vi "ReCalc_V2.00.vi"(3 "Berechnen":bool, 4 "Datenspeicher":T3={"Fahrzeugdaten"="mit filter hd 85§$", "Auto-Pfad"="26.04.2024 14:10|C:\\Users\\User\\Dropbox\\Prüfstand\\Kurven\\lui\\105\\beduesung", "Rolle [Inkr/U]"=200, "Rollenumfang [m]"=1.255, "Rollenträgheit [kgm²]"=9.1, "Zündung [Imp/U]"=2.0, "Getriebe [1:]"=7.93, "Reifenumfang [m] "=1.293, "Grossanzeige"=7.725, "Gl. Mittelwert"=25, "Differenzenquotient"=8, 1, "dT [s]"=0.0204081632653061, "Strecke [m]"=365.955776857143, "Lufttemperatur [°C]"=13.1, "Mv: n1 [1/min]"=1.0, "Luftdruck [mbar]"=899.6, "nRolle"=array[1261 elements], "nWelle"=array[1261 elements], "AFR"=array[1261 elements], "EGT"=array[1261 elements], "Übersetzung ermitteln aus"=2, "[s]"=3.0, "Mv: M0 [Nm]"=0.0, "Mv: M1 [Nm]"=0.0, "n vom Gas [1/min]"=8000.0, "dT ungefiltert [s]"=array[1261 elements], [], "Boolesch"=FALSE, "Serielle Schnittstelle"="COM13", "nKuWe/nRolle"=7.725, "v vom Gas [km/h]"=0.0}) -> ()   [LabVIEW 2014]
uses:
  <vilib>/Utility/miscctls.llb/LVPointTypeDef.ctl
  <vilib>/Analysis/3filter.llb/IIR Filter (DBL).vi
  <vilib>/Analysis/NI_AALBase.lvlib
panel:
  out "Fahrzeugdaten":string
  out "Ergebnis":string
  out "EGT [°C]":dbl format="%#.1f"
  out "AFR / l":dbl format="%#.1f"
  out "PM-Graph":cluster{dbl[], dbl[]}[](graph)
  in  "AFR, EGT":bool caption="Messung Klimadaten"
  in  "Lambda":bool caption="Messung Klimadaten"
  in  "Überschrift Leistungsdiagramm":string
  out "AFR,EGT-Graph":cluster{dbl[], "AFR":dbl[]}[](graph)
  out "Strecken":T1 {"Strecke7" scale=0.0..500.0; "Strecke6" scale=0.0..500.0; "Strecke5" scale=0.0..500.0; "Strecke4" scale=0.0..500.0; "Strecke3" scale=0.0..500.0; "Strecke2" scale=0.0..500.0; "Strecke1" max=600.0 scale=0.0..500.0}
  out "Dateiname":string
  out "Datum+Zeit":string="26.04.2024 14:10"
  out "Ereigniswert Überlagern":dbl=24.0
  in  "Mv: M1 [Nm]":dbl min=0.0
  in  "Mv: M0 [Nm]":dbl min=0.0
  in  "Mv: n1 [1/min]":u16=1 min=1
  out "Überlagerung":bool
  out "CursorY2 - Beschriftung":string="M [Nm]"
  out "CursorX - Beschriftung":string="n [1/min]"
  out "M [Nm]":dbl=4550.322600913994 format="%#.1f"
  out "P [PS]":dbl=3885.8131998402705 format="%#.1f"
  out "n [1/min]":dbl=5997.814814814815 caption="n {1/min]" format="%#.0f"
  in  "v vom Gas [km/h]":dbl
  in  "Legende":bool=TRUE
  in  "Überlagern":bool
  out "Übersetzung aus:":T2(ring)=enum."nKuWe / nRolle"
  in  "Speichern":bool
  out "Reifenumfang [m]":dbl=1.293
  out "Getriebe [1:]":dbl=7.93
  out "Zündung [Imp/U]":dbl=2.0
  out "Rollengeber [Inkr/U]":u16=200
  out "Luftdruck [mbar]":dbl=899.6
  out "Lufttemperatur [°C]":dbl=13.1
  in  "Stopp":bool
  in  "Rollenträgheit [kgm²]":dbl=9.1
  in  "Gl. Mittelwert":u8=25
  in  "Differenzenquotient":u8=8
  in  "n vom Gas [1/min]":dbl=8000.0
  out "Rollenumfang [m]":dbl=1.255 format="%.3f"
  out "nKuWe / nRolle":dbl=7.725 format="%.2f"
  in  "Drucken":bool
  out "Pmax":string
  in  "Öffnen":bool
  out "[s]":dbl=3.0
  # "AFR / l &  EGT"
  # "AFR <> l"
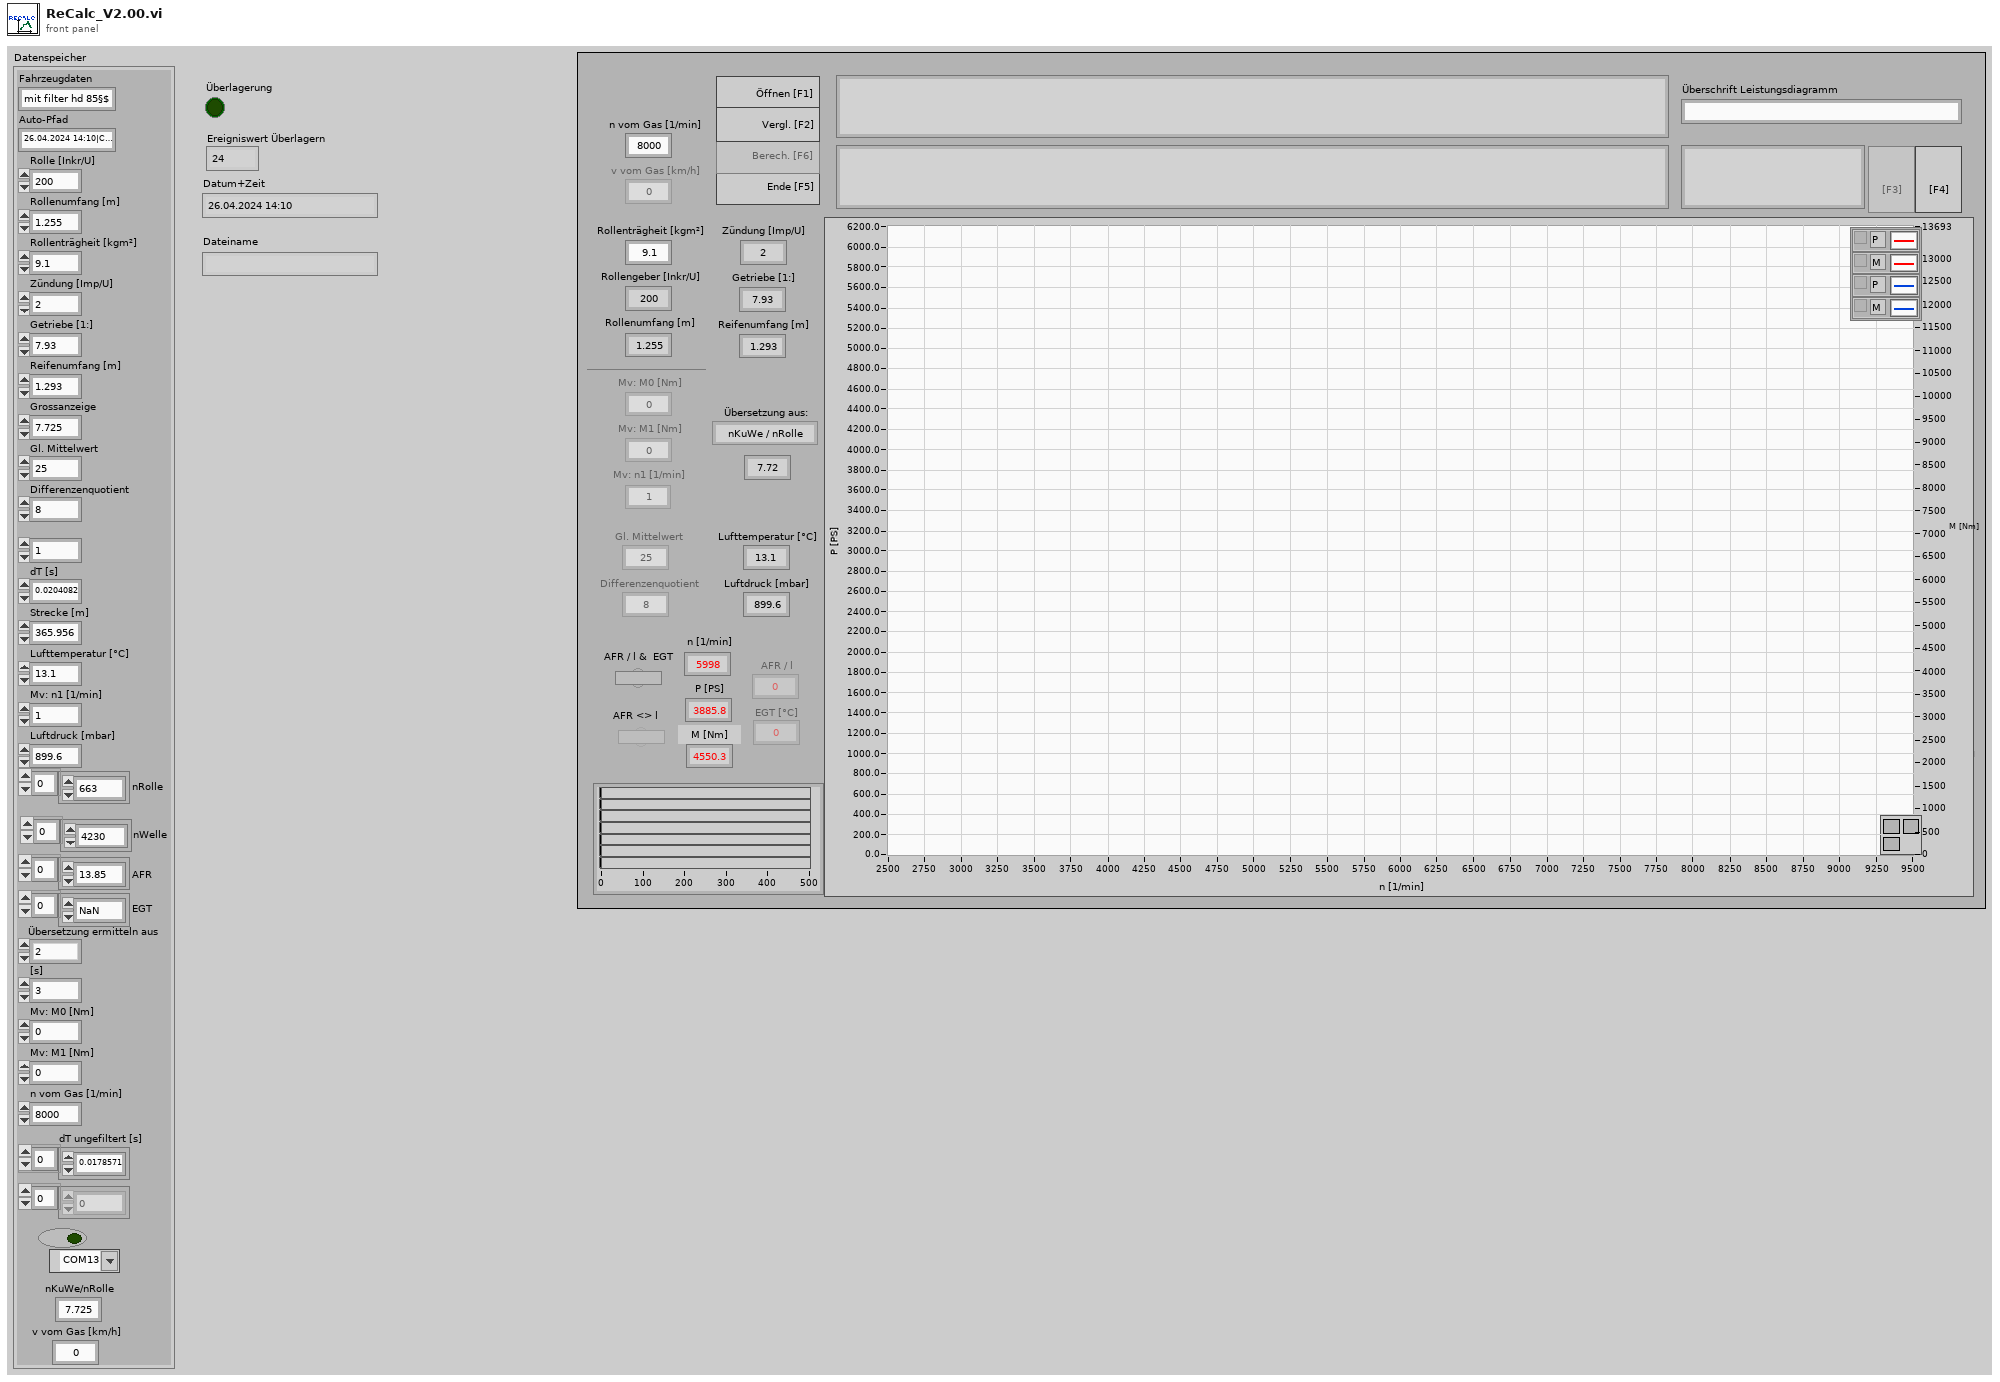
[diagram p1: front panel]
types:
  T1 = cluster{"Strecke1":dbl, "Strecke2":dbl, "Strecke3":dbl, "Strecke4":dbl, "Strecke5":dbl, "Strecke6":dbl, "Strecke7":dbl}
  T2 = enum8{"Zündsignal", "Getriebe & Reifen", "nKuWe / nRolle", "Vario [km/h]"}
  T3 = cluster{"Fahrzeugdaten":string, "Auto-Pfad":string, "Rolle [Inkr/U]":u16, "Rollenumfang [m]":dbl, "Rollenträgheit [kgm²]":dbl, "Zündung [Imp/U]":dbl, "Getriebe [1:]":dbl, "Reifenumfang [m] ":dbl, "Grossanzeige":dbl, "Gl. Mittelwert":u8, "Differenzenquotient":u8, u8, "dT [s]":dbl, "Strecke [m]":dbl, "Lufttemperatur [°C]":dbl, "Mv: n1 [1/min]":dbl, "Luftdruck [mbar]":dbl, "nRolle":dbl[], "nWelle":dbl[], "AFR":dbl[], "EGT":dbl[], "Übersetzung ermitteln aus":u8, "[s]":dbl, "Mv: M0 [Nm]":dbl, "Mv: M1 [Nm]":dbl, "n vom Gas [1/min]":dbl, "dT ungefiltert [s]":dbl[], i32[], "Boolesch":bool, "Serielle Schnittstelle":refnum<visa-resource-name>, "nKuWe/nRolle":dbl, "v vom Gas [km/h]":dbl}
  T4 = typedef "LVPointTypeDef.ctl" = cluster{"Horizontal":i16, "Vertical":i16}
  T5 = enum8{"Enabled", "Disabled", "Disabled and Grayed Out"}
  T6 = cluster{"Fahrzeugdaten":string, "Auto-Pfad":string, "Rolle [Inkr/U]":u16, "Rollenumfang [m]":dbl, "Rollenträgheit [kgm²]":dbl, "Zündung [Imp/U]":dbl, "Getriebe [1:]":dbl, "Reifenumfang [m] ":dbl, "Grossanzeige":dbl, "Gl. Mittelwert":u8, "Differenzenquotient":u8, "AFR,EGT":u8, "dT [s]":dbl, "Strecke [m]":dbl, "Lufttemperatur [°C]":dbl, "Mv: n1 [1/min]":dbl, "Luftdruck [mbar]":dbl, "nRolle":dbl[], "nWelle":dbl[], "AFR":dbl[], "EGT":dbl[], "Übersetzung ermitteln aus":u8, "[s]":dbl, "Mv: M0 [Nm]":dbl, "Mv: M1 [Nm]":dbl, "n vom Gas [1/min]":dbl, "dT-Array [s]":dbl[], i32[], "Boolesch":bool, "Serielle Schnittstelle":refnum<visa-resource-name>, "nKuWe/nRolle":dbl, "v vom Gas [km/h]":dbl}
  T7 = enum16{"Zündsignal", "Getriebe & Reifen", "nKuWe / nRolle", "Vario (km/h)"}
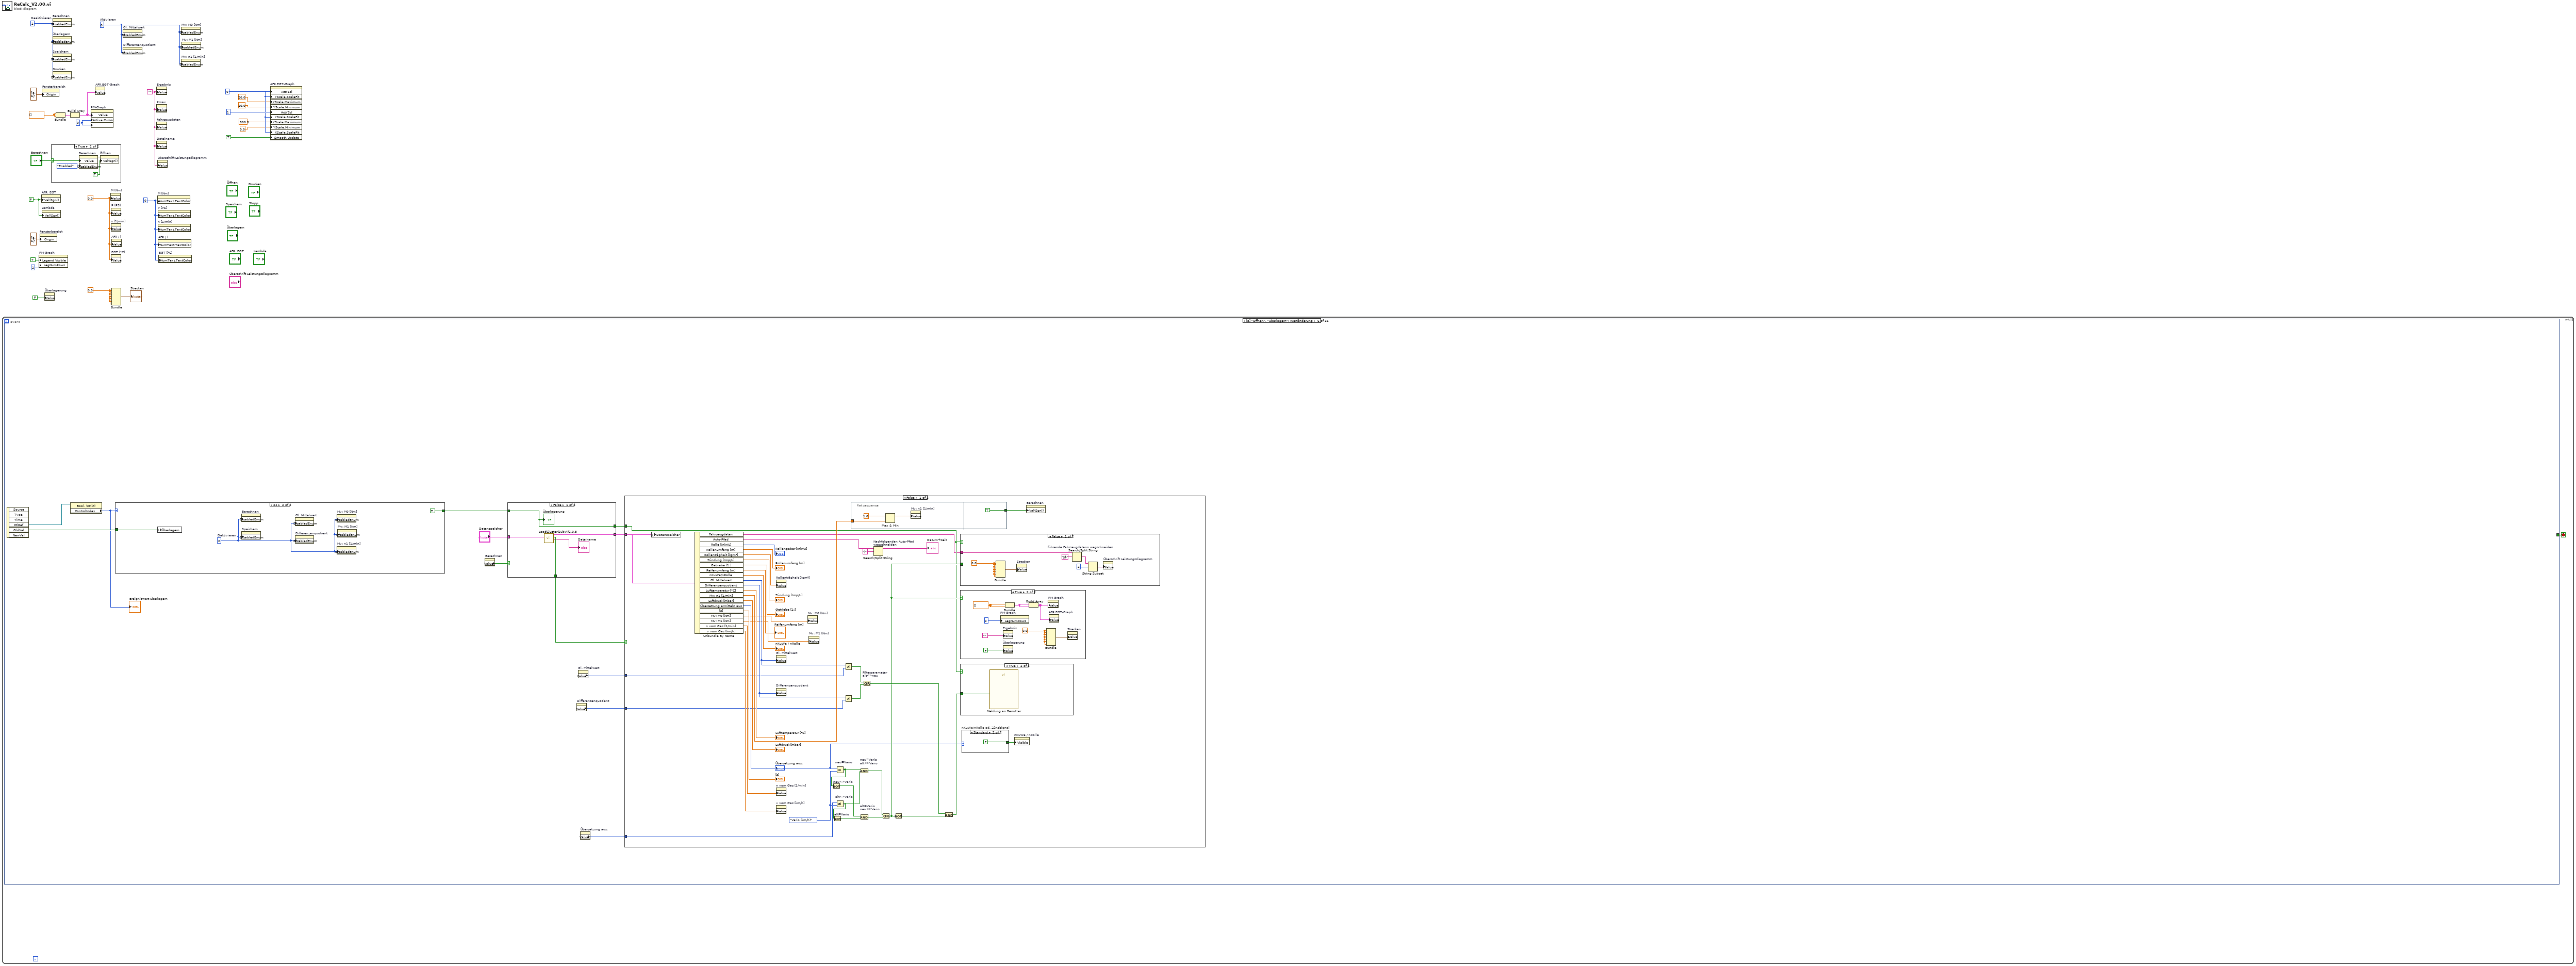
[diagram p0: block diagram]
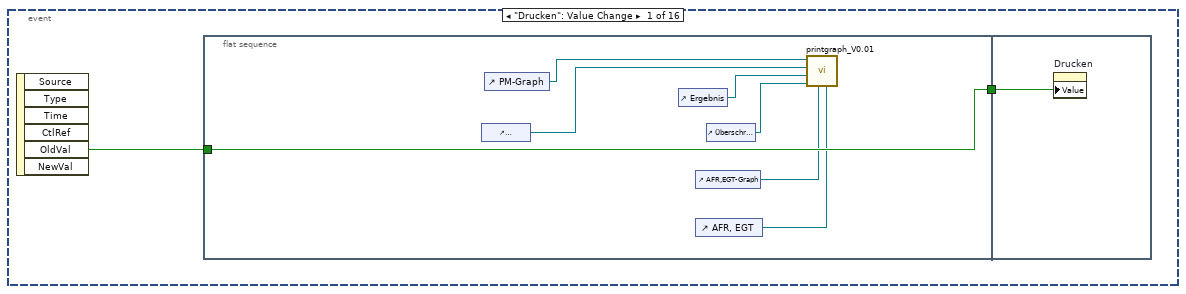
[diagram p3: hidden frame]
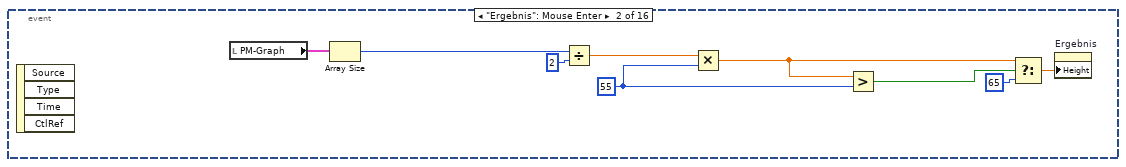
[diagram p4: hidden frame]
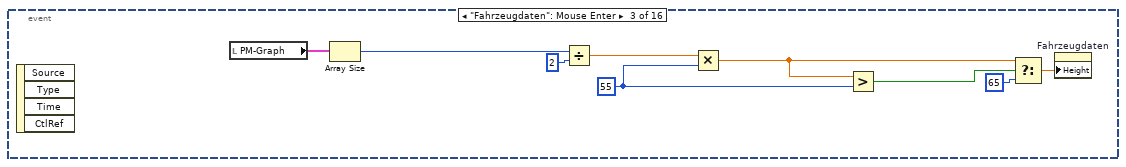
[diagram p5: hidden frame]
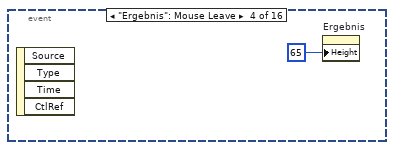
[diagram p6: hidden frame]
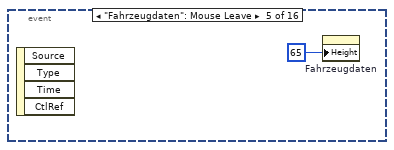
[diagram p7: hidden frame]
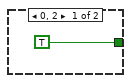
[diagram p8: hidden frame]
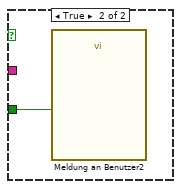
[diagram p10: hidden frame]
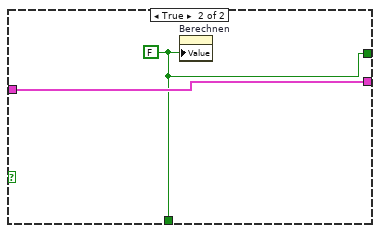
[diagram p13: hidden frame]
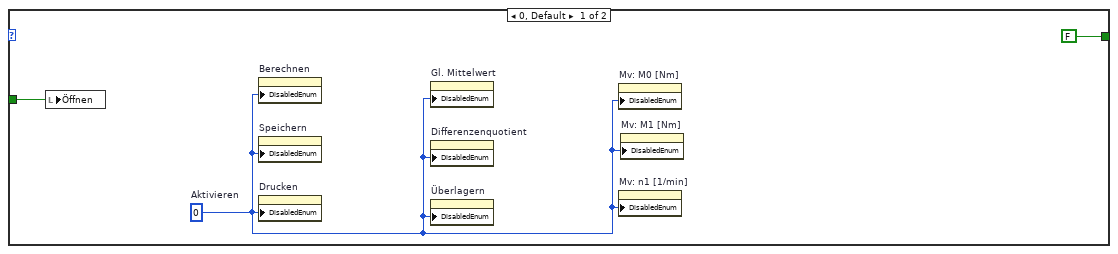
[diagram p14: hidden frame]
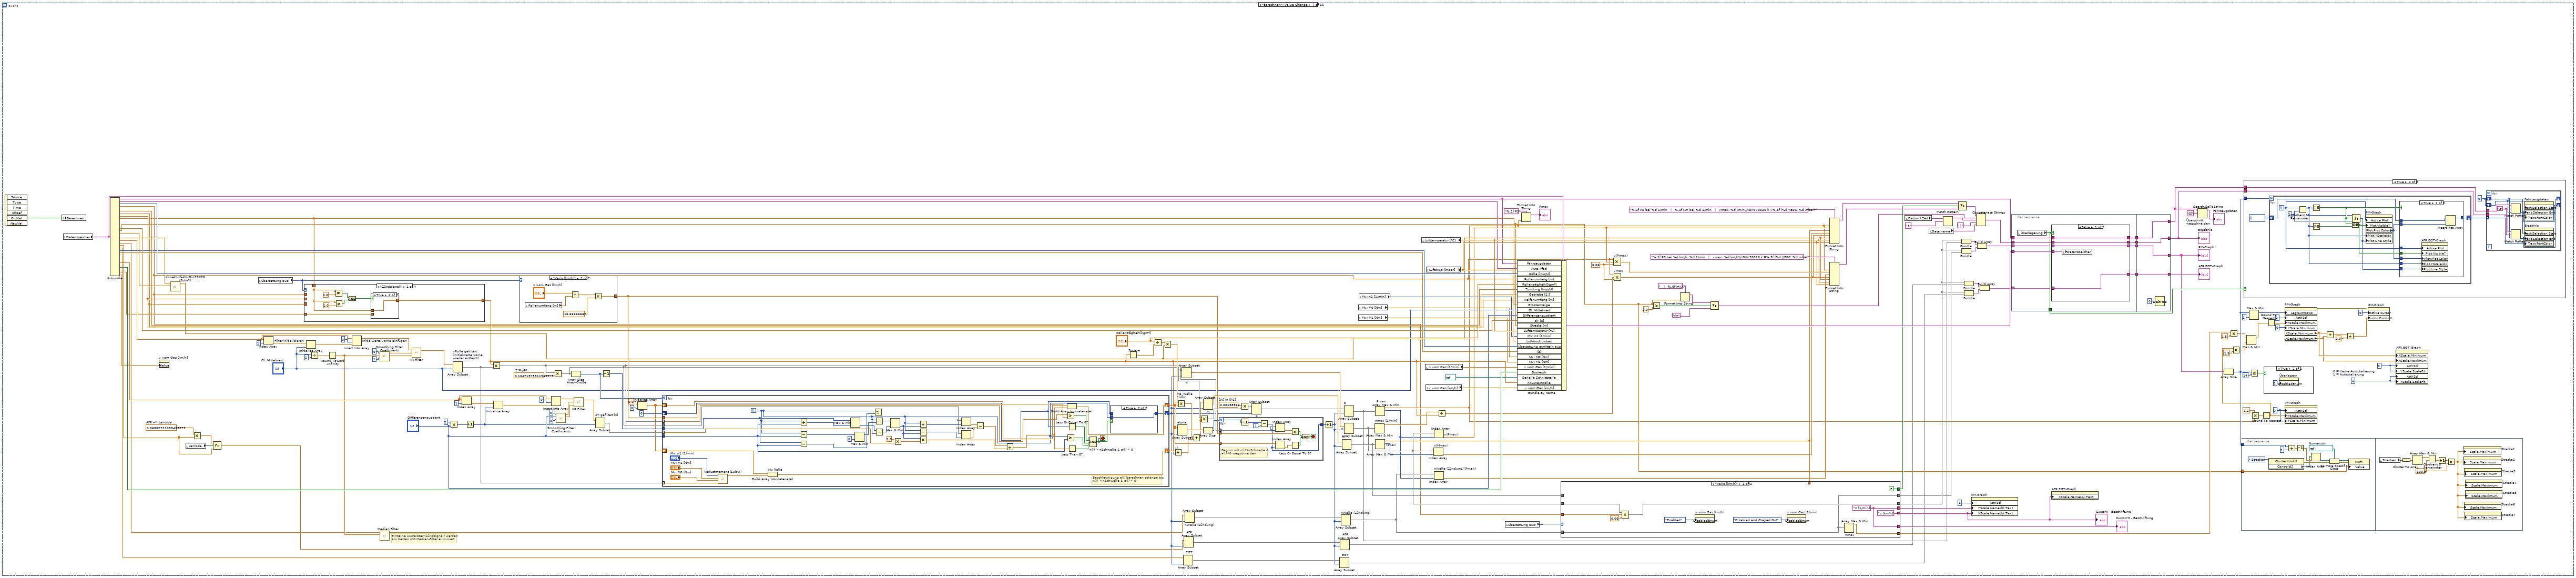
[diagram p15: hidden frame]
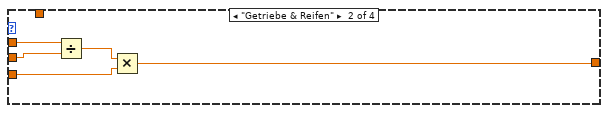
[diagram p17: hidden frame]
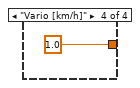
[diagram p19: hidden frame]
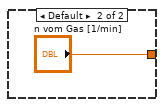
[diagram p20: hidden frame]
diagram:
  w6 = 0
  w10 = FALSE
  w14 = 0.0
  w18 = 0
  w12 = 0
  w11 = 0.0
  w19 = dbl[] []
  w16 = 0  # Aktivieren
  w22 = 2  # Deaktivieren
  w13 = ""
  n1 = while {
    stop <- w26 stop-if-true
    n2 = event shown="[5] \"Öffnen\", \"Überlagern\": Wertänderung" {
      selector: _ -> [_ _ _ _ _ _ _ _ _ _ _ _ _ _ _ _]
      dyn-events: _ -> [_ _ _ _ _ _ _ _ _ _ _ _ _ _ _ _]
      timeout: _ -> [_ _ _ _ _ _ _ _ _ _ _ _ _ _ _ _]
      tunnel: [_ _ _ _ _ _ _ _ w532 _ _ _ _ _ _ _] -> w26
      event "Drucken": Value Change {
        n3 = event-data() -> ("OldVal"=w28:bool)  [unwired: 1 in, 5 out]
        n4 = flat-sequence {
          tunnel: [w35] -> w27
          tunnel: w28 -> [w35]
          tunnel: w27 -> [w36]
          frame #0 {
            n5 = control-ref of="Fahrzeugdaten"() -> (w33:refnum<vi>)
            n6 = control-ref of="PM-Graph"() -> (w34:refnum<vi>)
            n7 = control-ref of="Ergebnis"() -> (w32:refnum<vi>)
            n8 = control-ref of="AFR,EGT-Graph"() -> (w30:refnum<vi>)
            n9 = control-ref of="AFR, EGT"() -> (w29:refnum<vi>)
            n10 = control-ref of="Überschrift Leistungsdiagramm"() -> (w31:refnum<vi>)
            n11 = call "printgraph_V0.01.vi"("AFR"=w29, "AFR-Graph (Eingang)"=w30, "Überschrift"=w31, "Ergebnis"=w32, "Fahrzeugdaten"=w33, "PM-Graph (Eingang)"=w34) -> ()  [unwired: 6 in]
          }
          frame #1 {
            n12 = property on="Drucken" class="Bool. (strikt)"("Value"=w36) -> ()  [unwired: 2 in, 2 out]
          }
        }
      }
      event "Ergebnis": Mouse Enter {
        w39 = u32 55 ("Größe:Höhe")
        n13 = event-data() -> ()  [unwired: 1 in, 4 out]
        n14 = local read "PM-Graph"() -> (w45:cluster{dbl[], dbl[]}[])
        n15 = Array Size(array=w45) -> (size(s)=w44:i32)
        n16 = Divide(x=w44, y=2) -> (x/y=w42:dbl)
        n17 = Multiply(x=w42, y=w39) -> (x*y=w40:dbl)
        n18 = Greater?(x=w40, y=w39) -> (0:w41:bool)
        n19 = Select(t=w40, s=w41, f=u32 65 ("Größe:Höhe")) -> (s? t:f=w38:dbl)
        n20 = property on="Ergebnis" class="Str"("Height"=w38) -> ()  [unwired: 2 in, 2 out]
      }
      event "Fahrzeugdaten": Mouse Enter {
        w48 = u32 55 ("Größe:Höhe")
        n21 = event-data() -> ()  [unwired: 1 in, 4 out]
        n22 = local read "PM-Graph"() -> (w54:cluster{dbl[], dbl[]}[])
        n23 = Array Size(array=w54) -> (size(s)=w53:i32)
        n24 = Divide(x=w53, y=2) -> (x/y=w51:dbl)
        n25 = Multiply(x=w51, y=w48) -> (x*y=w49:dbl)
        n26 = Greater?(x=w49, y=w48) -> (0:w50:bool)
        n27 = Select(t=w49, s=w50, f=u32 65 ("Größe:Höhe")) -> (s? t:f=w47:dbl)
        n28 = property on="Fahrzeugdaten" class="Str"("Height"=w47) -> ()  [unwired: 2 in, 2 out]
      }
      event "Ergebnis": Mouse Leave {
        n29 = event-data() -> ()  [unwired: 1 in, 4 out]
        n30 = property on="Ergebnis" class="Str"("Height"=u32 65 ("Größe:Höhe")) -> ()  [unwired: 2 in, 2 out]
      }
      event "Fahrzeugdaten": Mouse Leave {
        n31 = event-data() -> ()  [unwired: 1 in, 4 out]
        n32 = property on="Fahrzeugdaten" class="Str"("Height"=u32 65 ("Größe:Höhe")) -> ()  [unwired: 2 in, 2 out]
      }
      event "Öffnen", "Überlagern": Value Change {
        n33 = event-data() -> ("CtlRef"=w67:refnum<vi>, "OldVal"=w58:bool)  [unwired: 1 in, 4 out]
        n34 = property class="Bool. (strikt)"(reference=w67) -> ("ControlIndex"=w57:i32)  [unwired: 1 in, 2 out]
        "Ereigniswert Überlagern" <- w57
        n35 = case shown="24" w57 {
          tunnel: w58 -> [w143 w146]
          tunnel: [FALSE ("Überlagerung") TRUE ("Überlagerung")] -> w66
          frame 0, Default {
            w141 = 0  # Aktivieren
            n36 = local write "Öffnen"(w143) -> ()
            n37 = property on="Berechnen" class="Bool. (strikt)"("DisabledEnum"=w141) -> ()  [unwired: 2 in, 2 out]
            n38 = property on="Speichern" class="Bool. (strikt)"("DisabledEnum"=w141) -> ()  [unwired: 2 in, 2 out]
            n39 = property on="Drucken" class="Bool. (strikt)"("DisabledEnum"=w141) -> ()  [unwired: 2 in, 2 out]
            n40 = property on="Gl. Mittelwert" class="DigWert (strikt)"("DisabledEnum"=w141) -> ()  [unwired: 2 in, 2 out]
            n41 = property on="Differenzenquotient" class="DigWert (strikt)"("DisabledEnum"=w141) -> ()  [unwired: 2 in, 2 out]
            n42 = property on="Überlagern" class="Bool. (strikt)"("DisabledEnum"=w141) -> ()  [unwired: 2 in, 2 out]
            n43 = property on="Mv: M0 [Nm]" class="DigWert (strikt)"("DisabledEnum"=w141) -> ()  [unwired: 2 in, 2 out]
            n44 = property on="Mv: n1 [1/min]" class="DigWert (strikt)"("DisabledEnum"=w141) -> ()  [unwired: 2 in, 2 out]
            n45 = property on="Mv: M1 [Nm]" class="DigWert (strikt)"("DisabledEnum"=w141) -> ()  [unwired: 2 in, 2 out]
          }
          frame 24 {
            w144 = 2  # Dektivieren
            n46 = local write "Überlagern"(w146) -> ()
            n47 = property on="Berechnen" class="Bool. (strikt)"("DisabledEnum"=w144) -> ()  [unwired: 2 in, 2 out]
            n48 = property on="Speichern" class="Bool. (strikt)"("DisabledEnum"=w144) -> ()  [unwired: 2 in, 2 out]
            n49 = property on="Gl. Mittelwert" class="DigWert (strikt)"("DisabledEnum"=w144) -> ()  [unwired: 2 in, 2 out]
            n50 = property on="Differenzenquotient" class="DigWert (strikt)"("DisabledEnum"=w144) -> ()  [unwired: 2 in, 2 out]
            n51 = property on="Mv: M0 [Nm]" class="DigWert (strikt)"("DisabledEnum"=w144) -> ()  [unwired: 2 in, 2 out]
            n52 = property on="Mv: n1 [1/min]" class="DigWert (strikt)"("DisabledEnum"=w144) -> ()  [unwired: 2 in, 2 out]
            n53 = property on="Mv: M1 [Nm]" class="DigWert (strikt)"("DisabledEnum"=w144) -> ()  [unwired: 2 in, 2 out]
          }
        }
        n54 = property on="Berechnen" class="Bool. (strikt)"() -> ("Value"=w65:bool)  [unwired: 2 in, 2 out]
        n55 = case shown="False" w65 {
          tunnel: "Datenspeicher" -> [w137 w140]
          tunnel: w66 -> [w138 _]
          tunnel: [w136 w140] -> w63
          tunnel: [w138 w139] -> w64
          tunnel: [w135 w139] -> w62
          frame False {
            n56 = call "LoadCluster(SubVI)2.0.5.vi"("Datenspeicher"=w137) -> ("Dateiname"=→"Dateiname":string, "cancelled"=w135:bool, "Value"=w136:T6)  [unwired: 8 in]
            "Überlagerung" <- w138
          }
          frame True {
            w139 = FALSE
            n57 = property on="Berechnen" class="Bool. (strikt)"("Value"=w139) -> ()  [unwired: 2 in, 2 out]
          }
        }
        n58 = property on="Differenzenquotient" class="DigWert (strikt)"() -> ("Value"=w60:u8)  [unwired: 2 in, 2 out]
        n59 = property on="Gl. Mittelwert" class="DigWert (strikt)"() -> ("Value"=w59:u8)  [unwired: 2 in, 2 out]
        n60 = property on="Übersetzung aus:" class="Enum (strikt)"() -> ("Value"=w61:T2)  [unwired: 2 in, 2 out]
        n61 = case shown="False" w62 {
          tunnel: w64 -> [w88 _]
          tunnel: w63 -> [w90 _]
          tunnel: w61 -> [w81 _]
          tunnel: w60 -> [w80 _]
          tunnel: w59 -> [w79 _]
          frame False {
            w82 = T7."Vario (km/h)"
            n62 = local write "Datenspeicher"(w90) -> ()
            n63 = Unbundle By Name(w90) -> ("Fahrzeugdaten"=w71:string, "Auto-Pfad"=w74:string, "Rolle [Inkr/U]"=→"Rollengeber [Inkr/U]":u16, "Rollenumfang [m]"=→"Rollenumfang [m]":dbl, "Rollenträgheit [kgm²]"=w102:dbl, "Zündung [Imp/U]"=→"Zündung [Imp/U]":dbl, "Getriebe [1:]"=→"Getriebe [1:]":dbl, "Reifenumfang [m]"=→"Reifenumfang [m]":dbl, "nKuWe/nRolle"=→"nKuWe / nRolle":dbl, "Gl. Mittelwert"=w99:u8, "Differenzenquotient"=w98:u8, "Lufttemperatur [°C]"=→"Lufttemperatur [°C]":dbl, "Mv: n1 [1/min]"=w108:dbl, "Luftdruck [mbar]"=→"Luftdruck [mbar]":dbl, "Übersetzung ermitteln aus"=w70:u8, "[s]"=→"[s]":dbl, "Mv: M0 [Nm]"=w76:dbl, "Mv: M1 [Nm]"=w75:dbl, "n vom Gas [1/min]"=w110:dbl, "v vom Gas [km/h]"=w94:dbl)
            "Übersetzung aus:" <- w70
            n64 = property on="Rollenträgheit [kgm²]" class="DigWert (strikt)"("Value"=w102) -> ()  [unwired: 2 in, 2 out]
            n65 = property on="Gl. Mittelwert" class="DigWert (strikt)"("Value"=w99) -> ()  [unwired: 2 in, 2 out]
            n66 = property on="Differenzenquotient" class="DigWert (strikt)"("Value"=w98) -> ()  [unwired: 2 in, 2 out]
            n67 = property on="n vom Gas [1/min]" class="DigWert (strikt)"("Value"=w110) -> ()  [unwired: 2 in, 2 out]
            n68 = property on="v vom Gas [km/h]" class="DigWert (strikt)"("Value"=w94) -> ()  [unwired: 2 in, 2 out]
            n69 = property on="Mv: M0 [Nm]" class="DigWert (strikt)"("Value"=w76) -> ()  [unwired: 2 in, 2 out]
            n70 = property on="Mv: M1 [Nm]" class="DigWert (strikt)"("Value"=w75) -> ()  [unwired: 2 in, 2 out]
            n71 = Equal? "neu=Vario"(x=w70, y=w82) -> (x = y?=w83:bool)
            n72 = Not "neu<>Vario"(x=w83) -> (.not. x?=w84:bool)
            n73 = Not Equal? "alt<>Vario"(x=w81, y=w82) -> (x != y?=w77:bool)
            n74 = Not "alt=Vario"(x=w77) -> (.not. x?=w78:bool)
            n75 = Not Equal?(x=w99, y=w79) -> (x != y?=w97:bool)
            n76 = Not Equal?(x=w98, y=w80) -> (x != y?=w96:bool)
            n77 = flat-sequence {
              tunnel: w108 -> [w132]
              tunnel: [TRUE] -> w91
              frame #0 {
                n78 = Max & Min(x=1.0, y=w132) -> (max(x,y)=w130:dbl)  [unwired: 1 out]
                n79 = property on="Mv: n1 [1/min]" class="DigWert (strikt)"("Value"=w130) -> ()  [unwired: 2 in, 2 out]
              }
              frame #1 {
              }
            }
            n80 = And "neu=Vario\nalt<>Vario"(x=w83, y=w77) -> (x .and. y?=w86:bool)
            n81 = And "alt=Vario\nneu<>Vario"(x=w84, y=w78) -> (x .and. y?=w85:bool)
            n82 = Or "Filterparameter\nalt<>neu"(x=w97, y=w96) -> (x .or. y?=w92:bool)
            n83 = Search/Split String "Nachfolgenden Auto-Pfad wegschneiden"(string=w74, search string/char (-)="|") -> (substring before match=→"Datum+Zeit":string)  [unwired: 1 in, 2 out]
            n84 = Or(x=w86, y=w85) -> (x .or. y?=w89:bool)
            n85 = Not(x=w89) -> (.not. x?=w93:bool)
            n86 = And(x=w92, y=w93) -> (x .and. y?=w87:bool)
            n87 = case shown="True" w89 {
              frame False {
              }
              frame True {
                w116 = 0.0
                w117 = dbl[] []
                n88 = property on="PM-Graph" class="XYGraph (strikt)"("LegNumRows"=2) -> ()  [unwired: 2 in, 2 out]
                n89 = property on="Ergebnis" class="Str"("Value"="") -> ()  [unwired: 2 in, 2 out]
                n90 = property on="Überlagerung" class="Bool. (strikt)"("Value"=FALSE) -> ()  [unwired: 2 in, 2 out]
                n91 = Bundle(w117, w117) -> (w114:cluster{dbl[], dbl[]})  [unwired: 1 in]
                n92 = Build Array(w114, w114) -> (w113:cluster{dbl[], dbl[]}[])
                n93 = Bundle(w116, w116, w116, w116, w116, w116, w116) -> (w115:cluster{dbl, dbl, dbl, dbl, dbl, dbl, dbl})  [unwired: 1 in]
                n94 = property on="PM-Graph" class="XYGraph (strikt)"("Value"=w113) -> ()  [unwired: 2 in, 2 out]
                n95 = property on="AFR,EGT-Graph" class="XYGraph (strikt)"("Value"=w113) -> ()  [unwired: 2 in, 2 out]
                n96 = property on="Strecken" class="Cluster (strikt)"("Value"=w115) -> ()  [unwired: 2 in, 2 out]
              }
            }
            n97 = case shown="True" w88 {
              tunnel: w87 -> [_ w129]
              frame False {
              }
              frame True {
                n98 = call "Meldung an Benutzer"("Enable"=w129) -> ()  [unwired: 9 in, 2 out]
              }
            }
            n99 = case shown="False" w88 {
              tunnel: w89 -> [_ w128]
              tunnel: w71 -> [w121 _]
              frame False {
                w126 = 0.0
                n100 = Bundle(w126, w126, w126, w126, w126, w126, w126) -> (w127:cluster{dbl, dbl, dbl, dbl, dbl, dbl, dbl})  [unwired: 1 in]
                n101 = property on="Strecken" class="Cluster (strikt)"("Value"=w127) -> ()  [unwired: 2 in, 2 out]
                n102 = Search/Split String "führende Fahrzeugdatenn wegschneiden"(string=w121, search string/char (-)="§$") -> (match + rest of string=w124:string)  [unwired: 1 in, 2 out]
                n103 = String Subset(string=w124, offset (0)=2) -> (substring=w125:string)  [unwired: 1 in]
                n104 = property on="Überschrift Leistungsdiagramm" class="Str"("Value"=w125) -> ()  [unwired: 2 in, 2 out]
              }
              frame True {
                n105 = call "Meldung an Benutzer2"("Enable"=w128) -> ()  [unwired: 9 in, 2 out]
              }
            }
            n106 = case "nKuWe/nRolle od. Zündsignal" shown="Standard" w70 {
              tunnel: [TRUE FALSE] -> w69
              frame 0, 2 {
              }
              frame Default {
              }
            }
            n107 = property on="nKuWe / nRolle" class="DigWert (strikt)"("Visible"=w69) -> ()  [unwired: 2 in, 2 out]
            n108 = property on="Berechnen" class="Bool. (strikt)"("Val(Sgnl)"=w91) -> ()  [unwired: 2 in, 2 out]
          }
          frame True {
          }
        }
      }
      event "Berechnen": Value Change {
        w156 = 0.06802721088435375  # AFR --> Lambda
        w168 = 1  # 0 = Keine Autoskalierung 1 = Autoskalierung
        w169 = 0
        w226 = 0.06
        w180 = 0
        w329 = 0.00135962  # [W] in [PS]
        w335 = 0.10471975511965978  # 2*Pi/60
        # "Einzelne Ausreisser (Zündsignal) werden\nam besten mit Median-Filter eliminiert"
        n109 = event-data() -> ("OldVal"=w304:bool)  [unwired: 1 in, 5 out]
        n110 = local write "Berechnen"(w304) -> ()
        n111 = local read "Datenspeicher"() -> (w311:T3)
        n112 = Unbundle(w311) -> ("Fahrzeugdaten"=w189:string, "Auto-Pfad"=w217:string, "Rolle [Inkr/U]"=w310:u16, "Rollenumfang [m]"=w150:dbl, "Zündung [Imp/U]"=w307:dbl, "Getriebe [1:]"=w148:dbl, "Reifenumfang [m]"=w149:dbl, "Grossanzeige"=w147:dbl, "dT [s]"=w279:dbl, "Strecke [m]"=w190:dbl, "Lufttemperatur [°C]"=w203:dbl, "Luftdruck [mbar]"=w202:dbl, "nRolle"=w244:dbl[], "nWelle"=w233:dbl[], "AFR"=w154:dbl[], "EGT"=w162:dbl[], "Übersetzung ermitteln aus"=w245:u8, "[s]"=w305:dbl, "dT ungefiltert [s]"=w243:dbl[], "Boolesch"=w308:bool, "nKuWe/nRolle"=w151:dbl, "v vom Gas [km/h]"=w264:dbl)  [unwired: 10 out]
        n113 = property on="v vom Gas [km/h]" class="DigWert (strikt)"("Value"=w264) -> ()  [unwired: 2 in, 2 out]
        n114 = call "KorrekturfaktorDin70020 (SubVI).vi"("Lufttemperatur [°C]"=w203, "Luftdruck [mbar]"=w202) -> ("Korrekturfaktor"=w201:dbl)  [unwired: 9 in]
        n115 = local read "Lambda"() -> (w158:bool)
        n116 = Multiply(x=w156, y=w154) -> (x*y=w155:dbl[])
        n117 = Select(t=w155, s=w158, f=w154) -> (s? t:f=w157:dbl[])
        n118 = local read "Übersetzung aus:"() -> (w153:T2)
        n119 = Index Array "Filter initialisieren"(array=w244, index=1) -> (element=w315:dbl)
        n120 = case shown="\"Zündsignal\"" w153 {
          tunnel: [w340 w350 w355 1.0] -> w152
          tunnel: w151 -> [w341 _ w355 _]
          tunnel: w150 -> [_ w354 _ _]
          tunnel: w149 -> [_ w353 _ _]
          tunnel: w148 -> [_ w351 _ _]
          tunnel: w147 -> [w342 _ _ _]
          frame "Zündsignal" {
            n121 = Not Equal?(x=w342, y=0.0) -> (x != y?=w344:bool)
            n122 = Not Equal?(x=w342, y=1.0) -> (x != y?=w345:bool)
            n123 = And(x=w344, y=w345) -> (x .and. y?=w343:bool)
            n124 = case shown="True" w343 {
              tunnel: w342 -> [_ w349]
              tunnel: w341 -> [w348 _]
              tunnel: [w348 w349] -> w340
              frame False {
              }
              frame True {
              }
            }
          }
          frame "Getriebe & Reifen" {
            n125 = Divide(x=w354, y=w353) -> (x/y=w352:dbl)
            n126 = Multiply(x=w352, y=w351) -> (x*y=w350:dbl)
          }
          frame "nKuWe / nRolle" {
          }
          frame "Vario [km/h]" {
          }
        }
        n127 = Initialize Array(w315, "Gl. Mittelwert") -> (w316:dbl[])
        n128 = Divide(x="Gl. Mittelwert", y=2) -> (x/y=w337:dbl)
        n129 = Round Toward -Infinity(1:w337) -> (0:w235:dbl)
        n130 = Insert Into Array "Initialwerte vorne einfügen"(array=w244, index=0, new element=w316) -> (w242:dbl[])
        n131 = call <vilib>:"Smoothing Filter Coefficients.vi"("shape"=1, "half-width"=w235, "type"=0) -> ("forward coefficients"=w246:dbl[], "reverse coefficients"=w247:dbl[])  [unwired: 6 in, 1 out]
        n132 = call <vilib>:"Median Filter.vi"("left rank"=w235, "X"=w233) -> ("Filtered X"=w232:dbl[])  [unwired: 8 in, 1 out]
        n133 = call-poly <vilib>:"IIR Filter.vi"("Forward Coefficients"=w246, "Reverse Coefficients"=w247, "X"=w242) -> ("Filtered X"=w313:dbl[])  [unwired: 1 in, 1 out]
        n134 = Multiply(x=2, y="Differenzenquotient") -> (x*y=w287:i32)
        n135 = Array Subset "nRolle gefiltert\n(Initialwerte vorne \nwieder entfernt)"(array=w313, index="Gl. Mittelwert") -> (w213:dbl[])  [unwired: 1 in]
        n136 = Index Array(array=w243, index=1 ("Index")) -> (element=w285:dbl)
        n137 = Increment(x=w287) -> (x+1=w280:i32)
        n138 = Multiply(x=w152, y=w213) -> (x*y=w237:dbl[])
        n139 = Initialize Array(w285, w280) -> (w283:dbl[])
        n140 = case shown="\"Vario [km/h]\"" w153 {
          tunnel: [w379 "n vom Gas [1/min]"] -> w263
          frame "Vario [km/h]" {
            n141 = local read "Rollenumfang [m]"() -> (w380:dbl)
            n142 = Divide(x="v vom Gas [km/h]", y=w380) -> (x/y=w378:dbl)
            n143 = Multiply(x=w378, y=16.66666667) -> (x*y=w379:dbl)
          }
          frame Default {
          }
        }
        n144 = Insert Into Array(array=w243, index=0 ("Index"), new element=w283) -> (w282:dbl[])
        n145 = Multiply(x=w237, y=w335) -> (x*y=w275:dbl[])
        n146 = call <vilib>:"Smoothing Filter Coefficients.vi"("shape"=0, "half-width"="Differenzenquotient", "type"=0) -> ("forward coefficients"=w290:dbl[], "reverse coefficients"=w291:dbl[])  [unwired: 6 in, 1 out]
        n147 = Array Size "Array-Größe"(array=w275) -> (size(s)=w333:i32)
        n148 = call-poly <vilib>:"IIR Filter.vi"("Forward Coefficients"=w290, "Reverse Coefficients"=w291, "X"=w282) -> ("Filtered X"=w281:dbl[])  [unwired: 1 in, 1 out]
        n149 = Array Subset "dT gefiltert [s]"(array=w281, index=w280) -> (w241:dbl[])  [unwired: 1 in]
        n150 = Decrement(x=w333) -> (x-1=w334:i32)
        n151 = Initialize Array(0.0 ("y"), 0) -> (w212:dbl[])
        n152 = for {
          N: w333 -> [_]
          tunnel: "Differenzenquotient" -> [w508]
          tunnel: w275 -> [w497]
          tunnel: w334 -> [w507]
          shift-right: [w512] -> w276
          shift-left: w212 -> [w496]
          tunnel: w237 -> [w510] mode=indexing
          tunnel: w263 -> [w494]
          shift-right: [w501] -> w160
          shift-left: 0 -> [w493]
          tunnel: w241 -> [w498] mode=indexing
          tunnel: w213 -> [w492] mode=indexing
          shift-right: [w486] -> w211
          shift-left: w212 -> [w487]
          i -> [w495]
          stop <- w502 stop-if-true
          # "Beschleunigung a(i) berechnen solange bis\nn(i) > nSchwelle & a(i) < 0"
          n153 = call "Verlustmoment (SubVI).vi"("n [1/min"=w492, "Verlustmoment M0 [Nm] bei n = 0"="Mv: M0 [Nm]", "Verlustmoment M1 [Nm] bei n1"="Mv: M1 [Nm]", "Rollendrehzahl n1 [1/min]"="Mv: n1 [1/min]") -> ("Mv"=w488:dbl)  [unwired: 7 in]
          n154 = Build Array (concatenate) "Mv Rolle"(w487, w488) -> (w486:dbl[])
          n155 = Add(x=w495, y=w508) -> (x+y=w520:i32)
          n156 = Subtract(x=w495, y=w508) -> (x-y=w526:i32)
          n157 = Subtract(x=w507, y=w508) -> (x-y=w509:i32)
          n158 = Max & Min(x=w507, y=w520) -> (min(x,y)=w521:i32)  [unwired: 1 out]
          n159 = Max & Min(x=w526, y=0) -> (max(x,y)=w524:i32)  [unwired: 1 out]
          n160 = Less Or Equal?(x=w495, y=w509) -> ()  [unwired: 1 out]
          n161 = Subtract(x=w495, y=w524) -> (x-y=w523:i32)
          n162 = Subtract(x=w521, y=w495) -> (x-y=w522:i32)
          n163 = Max & Min(x=w523, y=w522) -> (min(x,y)=w514:i32)  [unwired: 1 out]
          n164 = Multiply(x=2.0, y=w498) -> (x*y=w499:dbl)
          n165 = Add(x=w495, y=w514) -> (x+y=w519:i32)
          n166 = Subtract(x=w495, y=w514) -> (x-y=w518:i32)
          n167 = Multiply(x=w514, y=w499) -> (x*y=w513:dbl)
          n168 = Index Array(array=w497, index=w519) -> (element=w516:dbl)
          n169 = Index Array(array=w497, index=w518) -> (element=w517:dbl)
          n170 = Subtract(x=w516, y=w517) -> (x-y=w515:dbl)
          n171 = Divide(x=w515, y=w513) -> (x/y=w506:dbl)
          n172 = Greater?(x=w510, y=w494) -> (0:w511:bool)
          n173 = Greater Or Equal?(x=w495, y=w508) -> (x >= y?=w505:bool)
          n174 = Build Array (concatenate)(w496, w506) -> (w512:dbl[])
          n175 = Less Or Equal To 0?(x=w493) -> (x <= 0?=w503:bool)
          n176 = Less Than 0?(x=w506) -> (x < 0?=w504:bool)
          n177 = Compound Arithmetic op=AND "n(i) > nSchwelle & a(i) < 0"(w504, w511, w503, w505) -> (w502:bool)
          n178 = case shown="True" w502 {
            tunnel: w495 -> [_ w528]
            tunnel: [w527 w528] -> w501
            tunnel: w493 -> [w527 _]
            frame False {
            }
            frame True {
            }
          }
        }
        n179 = Square(x=w152) -> (x^2=w330:dbl)
        n180 = Divide(x="Rollenträgheit [kgm²]", y=w330) -> (x/y=w327:dbl)
        n181 = Multiply(x=w327, y=w201) -> (x*y=w326:dbl)
        n182 = Divide ": i"(x=w211, y=w152) -> (x/y=w210:dbl[])
        n183 = Multiply "Ma_Welle\n* korr"(x=w276, y=w326) -> (x*y=w208:dbl[])
        n184 = Array Subset "alpha"(array=w276, length=w160) -> (w324:dbl[])  [unwired: 1 in]
        n185 = Array Subset "n"(array=w237, length=w160) -> (w240:dbl[])  [unwired: 1 in]
        n186 = Array Subset "EGT"(array=w162, length=w160) -> (w164:dbl[])  [unwired: 1 in]
        n187 = Array Subset "AFR"(array=w157, length=w160) -> (w165:dbl[])  [unwired: 1 in]
        n188 = Array Subset "nWelle (Zündung)"(array=w232, length=w160) -> (w236:dbl[])  [unwired: 1 in]
        n189 = Add(x=w208, y=w210) -> (x+y=w209:dbl[])
        n190 = Multiply(x=w275, y=w209) -> (x*y=w328:dbl[])
        n191 = Array Subset "M"(array=w209, length=w160) -> (w278:dbl[])  [unwired: 1 in]
        n192 = Array Size(array=w324) -> (size(s)=w238:i32)
        n193 = for {
          N: w238 -> [w485]
          tunnel: w276 -> [w482]
          tunnel: w237 -> [w481]
          tunnel: w263 -> [w480]
          tunnel: [w478] -> w322
          i -> [w474]
          stop <- w479 stop-if-true
          # "Beginn mit n(i)<nSchwelle &  a(i)<0 wegschneiden"
          n194 = Decrement(x=w485) -> (x-1=w484:i32)
          n195 = Subtract(x=w484, y=w474) -> (x-y=w478:i32)
          n196 = Index Array(array=w481, index=w478) -> (element=w475:dbl)
          n197 = Index Array(array=w482, index=w478) -> (element=w483:dbl)
          n198 = Less?(x=w475, y=w480) -> (x < y?=w476:bool)
          n199 = Less Or Equal To 0?(x=w483) -> (x <= 0?=w477:bool)
          n200 = And(x=w476, y=w477) -> (x .and. y?=w479:bool)
        }
        n201 = Multiply(x=w329, y=w328) -> (x*y=w323:dbl[])
        n202 = Array Subset "P"(array=w323, length=w160) -> (w277:dbl[])  [unwired: 1 in]
        n203 = Increment(x=w322) -> (x+1=w163:i32)
        n204 = Array Subset "EGT"(array=w164, index=w163) -> (w159:dbl[])  [unwired: 1 in]
        n205 = Array Subset "AFR"(array=w165, index=w163) -> (w161:dbl[])  [unwired: 1 in]
        n206 = Array Subset "nWelle (Zündung)"(array=w236, index=w163) -> (w224:dbl[])  [unwired: 1 in]
        n207 = Array Subset "M"(array=w278, index=w163) -> (w267:dbl[])  [unwired: 1 in]
        n208 = Array Subset "P"(array=w277, index=w163) -> (w166:dbl[])  [unwired: 1 in]
        n209 = Array Subset "n"(array=w240, index=w163) -> (w239:dbl[])  [unwired: 1 in]
        n210 = local read "Mv: M0 [Nm]"() -> (w216:dbl)
        n211 = local read "Mv: M1 [Nm]"() -> (w215:dbl)
        n212 = local read "Mv: n1 [1/min]"() -> (w214:u16)
        n213 = Array Max & Min "nmax [1/min]"(array=w239) -> (max value=w306:dbl)  [unwired: 3 out]
        n214 = Array Max & Min "Pmax"(array=w166) -> (max value=w184:dbl, max index (indices)=w225:i32)  [unwired: 2 out]
        n215 = Array Max & Min "Mmax"(array=w267) -> (max value=w222:dbl, max index (indices)=w260:i32)  [unwired: 2 out]
        n216 = local read "Lufttemperatur [°C]"() -> (w219:dbl)
        n217 = local read "n vom Gas [1/min]"() -> (w266:dbl)
        n218 = local read "v vom Gas [km/h]"() -> (w265:dbl)
        n219 = local read "Luftdruck [mbar]"() -> (w218:dbl)
        n220 = Index Array "n(Mmax)"(array=w239, index=w260) -> (element=w221:dbl)
        n221 = Index Array "n(Pmax)"(array=w239, index=w225) -> (element=w228:dbl)
        n222 = Index Array "nWelle (Zündung) (Pmax)"(array=w224, index=w225) -> (element=w223:dbl)
        n223 = Divide(x=w306, y=w152) -> (x/y=w227:dbl)
        n224 = local read "Übersetzung aus:"() -> (w272:T2)
        n225 = Bundle By Name(cluster=w311, "Fahrzeugdaten"=w189, "Auto-Pfad"=w217, "Rolle [Inkr/U]"=w310, "Rollenumfang [m]"=w150, "Rollenträgheit [kgm²]"="Rollenträgheit [kgm²]", "Zündung [Imp/U]"=w307, "Getriebe [1:]"=w148, "Reifenumfang [m]"=w149, "Grossanzeige"=w147, "Gl. Mittelwert"="Gl. Mittelwert", "Differenzenquotient"="Differenzenquotient", "dT [s]"=w279, "Strecke [m]"=w190, "Lufttemperatur [°C]"=w219, "Mv: n1 [1/min]"=w214, "Luftdruck [mbar]"=w218, "Übersetzung ermitteln aus"=w245, "[s]"=w305, "Mv: M0 [Nm]"=w216, "Mv: M1 [Nm]"=w215, "n vom Gas [1/min]"=w266, "Boolesch"=w308, "Serielle Schnittstelle"=refnum<visa-resource-name> refnum, "nKuWe/nRolle"=w152, "v vom Gas [km/h]"=w265) -> (w303:T3)
        n226 = Format Into String(format string="%.1f PS" ("Format-String"), w184) -> (resulting string=→"Pmax":string)  [unwired: 2 in, 1 out]
        n227 = case shown="\"Vario [km/h]\"" w272 {
          tunnel: w150 -> [_ w399]
          tunnel: w239 -> [w389 w398]
          tunnel: [w389 w395] -> w170
          tunnel: [TRUE FALSE] -> w268
          tunnel: ["n [1/min]" "v [km/h]"] -> w176
          tunnel: w267 -> [w386 _]
          tunnel: [w386 w391] -> w167
          tunnel: [w382 w390] -> w250
          tunnel: w224 -> [_ w391]
          tunnel: [w383 w392] -> w249
          tunnel: w222 -> [w383 _]
          tunnel: [w382 w390] -> w248
          frame Default {
            w382 = "M [Nm]"
            n228 = property on="n vom Gas [1/min]" class="DigWert (strikt)"("DisabledEnum"=T5."Enabled" ("Deaktiviert")) -> ()  [unwired: 2 in, 2 out]
            n229 = property on="v vom Gas [km/h]" class="DigWert (strikt)"("DisabledEnum"=T5."Disabled and Grayed Out" ("Deaktiviert")) -> ()  [unwired: 2 in, 2 out]
          }
          frame "Vario [km/h]" {
            w390 = "n [1/min]"
            n230 = Compound Arithmetic op=MULTIPLY(w398, w399, 0.06) -> (w395:dbl[])
            n231 = property on="v vom Gas [km/h]" class="DigWert (strikt)"("DisabledEnum"=T5."Enabled" ("Deaktiviert")) -> ()  [unwired: 2 in, 2 out]
            n232 = property on="n vom Gas [1/min]" class="DigWert (strikt)"("DisabledEnum"=T5."Disabled and Grayed Out" ("Deaktiviert")) -> ()  [unwired: 2 in, 2 out]
            n233 = Array Max & Min "nmax"(array=w391) -> (max value=w392:dbl)  [unwired: 3 out]
          }
        }
        "CursorX - Beschriftung" <- w176
        "CursorY2 - Beschriftung" <- w248
        n234 = Compound Arithmetic op=MULTIPLY "v(Pmax)"(w150, w228, w226) -> (w270:dbl)
        n235 = Compound Arithmetic op=MULTIPLY "vmax"(w150, w227, w226) -> (w220:dbl)
        n236 = Greater?(x=w190, y=2.0) -> (0:w199:bool)
        n237 = Format Into String(format string="   |   %.0f m\\n" ("Format-String"), w190) -> (resulting string=w197:string)  [unwired: 2 in, 1 out]
        n238 = Select(t=w197, s=w199, f="\r\n") -> (s? t:f=w193:string)
        n239 = Format Into String(format string="%.1f PS bei %d 1/min   |   %.1f Nm bei %d 1/min   |   vmax: %d km/h\\nDIN 70020 k =%.3f (%d \\B0C, %d mbar)" ("Format-String"), w184, w228, w222, w221, w220, w201, w219, w218) -> (resulting string=w229:string)  [unwired: 2 in, 1 out]
        n240 = Format Into String(format string="%.1f PS bei %d km/h, %d 1/min   |   vmax: %d km/h\\nDIN 70020 k =%.3f (%d \\B0C, %d mbar)" ("Format-String"), w184, w270, w223, w220, w201, w219, w218) -> (resulting string=w230:string)  [unwired: 2 in, 1 out]
        n241 = local read "Datum+Zeit"() -> (w205:string)
        n242 = local read "Dateiname"() -> (w196:string)
        n243 = Match Pattern(string=w205, regular expression=" $") -> (before substring=w194:string)  [unwired: 1 in, 3 out]
        n244 = Select(t=w229, s=w268, f=w230) -> (s? t:f=w207:string)
        n245 = Bundle(w170, w166) -> (w297:cluster{dbl[], dbl[]})  [unwired: 1 in]
        n246 = Bundle(w170, w167) -> (w296:cluster{dbl[], dbl[]})  [unwired: 1 in]
        n247 = Bundle(w170, w161) -> (w173:cluster{dbl[], dbl[]})  [unwired: 1 in]
        n248 = Bundle(w170, w159) -> (w172:cluster{dbl[], dbl[]})  [unwired: 1 in]
        n249 = property on="PM-Graph" class="XYGraph (strikt)"("ActYScl"=1, "YScale.NameLbl.Text"=w250, "XScale.NameLbl.Text"=w176) -> ()  [unwired: 2 in, 2 out]
        n250 = Concatenate Strings(w207, w193, w194, " | ", w196) -> (w206:string)
        n251 = Build Array(w297, w296) -> (w258:cluster{dbl[], dbl[]}[])
        n252 = Build Array(w173, w172) -> (w171:cluster{dbl[], dbl[]}[])
        n253 = flat-sequence {
          tunnel: [w406] -> w302
          tunnel: [w409] -> w300
          tunnel: [w408] -> w299
          tunnel: w258 -> [w405]
          tunnel: [w404] -> w257
          tunnel: w189 -> [w407]
          tunnel: w303 -> [w410]
          tunnel: w206 -> [w411]
          tunnel: [w403] -> w175
          tunnel: w171 -> [w402]
          tunnel: [w434] -> w187
          tunnel: [w435] -> w301
          tunnel: w300 -> [w435]
          tunnel: w299 -> [w434]
          tunnel: [w432] -> w256
          tunnel: w257 -> [w432]
          tunnel: w175 -> [w431]
          tunnel: [w431] -> w174
          frame #0 {
            n254 = local read "Überlagerung"() -> (w406:bool)
            n255 = case shown="False" w406 {
              tunnel: w411 -> [w416 w429]
              tunnel: [w416 w430] -> w409
              tunnel: w410 -> [w415 _]
              tunnel: w407 -> [w414 w427]
              tunnel: [w414 w426] -> w408
              tunnel: w405 -> [w413 w421]
              tunnel: [w413 w420] -> w404
              tunnel: w402 -> [w412 w418]
              tunnel: [w412 w417] -> w403
              frame False {
                n256 = local write "Datenspeicher"(w415) -> ()
              }
              frame True {
                w425 = "\t"
                w428 = "\n"
                n257 = local read "Fahrzeugdaten"() -> (w424:string)
                n258 = local read "AFR,EGT-Graph"() -> (w419:cluster{dbl[], "AFR":dbl[]}[])
                n259 = local read "PM-Graph"() -> (w422:cluster{dbl[], dbl[]}[])
                n260 = local read "Ergebnis"() -> (w423:string)
                n261 = Concatenate Strings(w424, w425, w428, w427) -> (w426:string)
                n262 = Concatenate Strings(w423, w425, w428, w429) -> (w430:string)
                n263 = Insert Into Array(array=w422, new element=w421) -> (w420:cluster{dbl[], dbl[]}[])  [unwired: 1 in]
                n264 = Insert Into Array(array=w419, new element=w418) -> (w417:cluster{dbl[], "AFR":dbl[]}[])  [unwired: 1 in]
              }
            }
          }
          frame #1 {
            n265 = Wait (ms)(milliseconds to wait=u32 0 ("Zu wartende ms")) -> ()  [unwired: 1 out]
          }
        }
        n266 = property on="AFR,EGT-Graph" class="XYGraph (strikt)"("XScale.NameLbl.Text"=w176) -> ()  [unwired: 2 in, 2 out]
        n267 = Search/Split String "Überschrift wegschneiden"(string=w187, search string/char (-)="§$") -> (substring before match=→"Fahrzeugdaten":string)  [unwired: 1 in, 2 out]
        n268 = Array Size(array=w256) -> (size(s)=w191:i32)
        n269 = Multiply(x=w249, y=1.8) -> (x*y=w183:dbl)
        n270 = flat-sequence {
          tunnel: w191 -> [w367]
          tunnel: w190 -> [w358]
          frame #0 {
            w361 = refnum<vi> refnum  # Numerisch
            n271 = control-ref of="Strecken"() -> (w364:refnum<vi>)
            n272 = property on="Eigenschaftsknoten" class="Cluster (strikt)"(reference=w364) -> (error out=w362:errorcluster, "Controls[]"=w357:refnum<vi>[])  [unwired: 1 in, 1 out]
            n273 = Divide(x=w367, y=2) -> (x/y=w366:dbl)
            n274 = Decrement(x=w366) -> (x-1=w365:dbl)
            n275 = Index Array(array=w357, index=w365) -> (element=w363:refnum<vi>)
            n276 = To More Specific Class(target class=w361, reference=w363, error in=w362) -> (specific class reference=w360:refnum<vi>, error out=w359:errorcluster)
            n277 = property class="Num"(reference=w360, error in=w359, "Value"=w358) -> ()  [unwired: 2 out]
          }
          frame #1 {
            w370 = 100.0
            n278 = local read "Strecken"() -> (w375:T1)
            n279 = Cluster To Array(cluster=w375) -> (array=w374:dbl[])
            n280 = Array Max & Min(array=w374) -> (max value=w373:dbl)  [unwired: 3 out]
            n281 = Quotient & Remainder(x=w373, y=w370) -> (floor(x/y)=w372:dbl)  [unwired: 1 out]
            n282 = Increment(x=w372) -> (x+1=w371:dbl)
            n283 = Multiply(x=w371, y=w370) -> (x*y=w369:dbl)
            n284 = property on="Strecke1" class="Schieber (strikt)"("Scale.Maximum"=w369) -> ()  [unwired: 2 in, 2 out]
            n285 = property on="Strecke2" class="Schieber (strikt)"("Scale.Maximum"=w369) -> ()  [unwired: 2 in, 2 out]
            n286 = property on="Strecke6" class="Schieber (strikt)"("Scale.Maximum"=w369) -> ()  [unwired: 2 in, 2 out]
            n287 = property on="Strecke3" class="Schieber (strikt)"("Scale.Maximum"=w369) -> ()  [unwired: 2 in, 2 out]
            n288 = property on="Strecke7" class="Schieber (strikt)"("Scale.Maximum"=w369) -> ()  [unwired: 2 in, 2 out]
            n289 = property on="Strecke4" class="Schieber (strikt)"("Scale.Maximum"=w369) -> ()  [unwired: 2 in, 2 out]
            n290 = property on="Strecke5" class="Schieber (strikt)"("Scale.Maximum"=w369) -> ()  [unwired: 2 in, 2 out]
          }
        }
        n291 = case shown="True" w302 {
          tunnel: w191 -> [_ w446]
          tunnel: w301 -> [_ w443]
          tunnel: w187 -> [_ w442]
          frame False {
            w436 = TRUE ("Plot.Sichtbar")
            w440 = u32 16711680
            n292 = property on="Fahrzeugdaten" class="Str"("Text.Font:Color"=w440) -> ()  [unwired: 2 in, 2 out]
            n293 = property on="Ergebnis" class="Str"("Text.Font:Color"=w440) -> ()  [unwired: 2 in, 2 out]
            n294 = property on="PM-Graph" class="XYGraph (strikt)"("Active Plot"=0, "Plot.Visible?"=w436, "Active Plot"=1, "Plot.Visible?"=w436) -> ()  [unwired: 2 in, 2 out]
            n295 = property on="AFR,EGT-Graph" class="XYGraph (strikt)"("Active Plot"=0, "Plot.Visible?"=w436) -> ()  [unwired: 2 in, 2 out]
          }
          frame True {
            w441 = 0
            n296 = for {
              N: w446 -> [_]
              shift-right: [w464] -> w444
              shift-left: u32[] [] -> [w463]
              i -> [w459]
              w462 = 2 ("y")
              n297 = Quotient & Remainder(x=w459, y=w462) -> (x-y*floor(x/y)=w456:i32)  [unwired: 1 out]
              n298 = Equal To 0?(x=w456) -> (x = 0?=w460:bool)
              n299 = Not Equal To 0?(x=w456) -> (x != 0?=w461:bool)
              n300 = Or(x=w460, y=w461) -> (x .or. y?=w458:bool)
              n301 = Select(t=w456, s=w460, f=w462) -> (s? t:f=w455:i32)
              n302 = property on="PM-Graph" class="XYGraph (strikt)"("Active Plot"=w459, "Plot.Visible?"=w458, "Plot.YScaleIdx"=w456, "Plot.Line Style"=w455) -> ("Plot.Plot Color"=w457:u32)  [unwired: 2 in, 2 out]
              n303 = case shown="True" w460 {
                tunnel: w457 -> [_ w473]
                tunnel: [w465 w472] -> w464
                tunnel: w463 -> [w465 w471]
                tunnel: w459 -> [_ w470]
                tunnel: w458 -> [_ w469]
                tunnel: w457 -> [_ w468]
                tunnel: w456 -> [_ w467]
                tunnel: w455 -> [_ w466]
                frame False {
                }
                frame True {
                  n304 = property on="AFR,EGT-Graph" class="XYGraph (strikt)"("Active Plot"=w470, "Plot.Visible?"=w469, "Plot.Plot Color"=w468, "Plot.YScaleIdx"=w467, "Plot.Line Style"=w466) -> ()  [unwired: 2 in, 2 out]
                  n305 = Insert Into Array(array=w471, new element=w473) -> (w472:u32[])  [unwired: 1 in]
                }
              }
            }
            n306 = for {
              shift-right: [w454] -> _
              shift-left: w441 -> [w451]
              tunnel: w444 -> [w452] mode=indexing
              tunnel: w443 -> [w453]
              tunnel: w442 -> [w450]
              shift-right: [w449] -> _
              shift-left: w441 -> [w448]
              w447 = "\t"
              n307 = Match Pattern(string=w450, regular expression=w447, offset (0)=w448) -> (offset past match=w449:i32)  [unwired: 3 out]
              n308 = Match Pattern(string=w453, regular expression=w447, offset (0)=w451) -> (offset past match=w454:i32)  [unwired: 3 out]
              n309 = property on="Fahrzeugdaten" class="Str"("Text.Selection Start"=w448, "Text.Selection End"=w449, "Text.FontColor"=w452) -> ()  [unwired: 2 in, 2 out]
              n310 = property on="Ergebnis" class="Str"("Text.Selection Start"=w451, "Text.Selection End"=w454, "Text.FontColor"=w452) -> ()  [unwired: 2 in, 2 out]
            }
          }
        }
        n311 = Max & Min(x=w191, y=2) -> (max(x,y)=w259:i32)  [unwired: 1 out]
        n312 = Greater Or Equal?(x=w191, y=14) -> (x >= y?=w294:bool)
        n313 = Multiply(x=w184, y=1.2) -> (x*y=w274:dbl)
        n314 = Round To Nearest(number=w274) -> (nearest integer value=w179:dbl)
        n315 = Multiply(x=w179, y=1.9) -> (x*y=w182:dbl)
        n316 = Max & Min(x=w183, y=w182) -> (max(x,y)=w181:dbl)  [unwired: 1 out]
        n317 = case shown="True" w294 {
          frame False {
          }
          frame True {
            n318 = property on="Überlagern" class="Bool. (strikt)"("DisabledEnum"=2) -> ()  [unwired: 2 in, 2 out]
          }
        }
        n319 = Round To Nearest(number=w181) -> (nearest integer value=w261:dbl)
        n320 = property on="PM-Graph" class="XYGraph (strikt)"("LegNumRows"=w259, "ActYScl"=1, "YScale.Maximum"=w261, "YScale.Minimum"=0) -> (error out=w253:errorcluster, "XScale.Minimum"=w178:dbl, "XScale.Maximum"=w177:dbl)  [unwired: 2 in, 1 out]
        n321 = property on="PM-Graph" class="XYGraph (strikt)"("ActYScl"=w180, "YScale.Maximum"=w179, "YScale.Minimum"=w180) -> ()  [unwired: 2 in, 2 out]
        n322 = Add(x=w178, y=w177) -> (x+y=w255:dbl)
        n323 = Divide(x=w255, y=2.0) -> (x/y=w252:dbl)
        n324 = property on="PM-Graph" class="XYGraph (strikt)"(error in=w253, "Active Cursor"=0, "Cursor.Cursor X"=w252) -> ()  [unwired: 1 in, 2 out]
        n325 = property on="AFR,EGT-Graph" class="XYGraph (strikt)"("XScale.Minimum"=w178, "XScale.Maximum"=w177, "ActYScl"=w169, "YScale.ScaleFit"=w169, "ActYScl"=w168, "YScale.ScaleFit"=w168) -> ()  [unwired: 2 in, 2 out]
        "Ergebnis" <- w301
        "PM-Graph" <- w256
        "AFR,EGT-Graph" <- w174
      }
      event "Speichern": Value Change {
        n326 = event-data() -> ("OldVal"=w530:bool)  [unwired: 1 in, 5 out]
        n327 = local write "Speichern"(w530) -> ()
        n328 = control-ref of="Datenspeicher"() -> (w529:refnum<vi>)
        n329 = call "SaveCluster.vi"("Datenspeicher"=w529) -> ()  [unwired: 1 in, 1 out]
      }
      event "Stopp": Value Change {
        n330 = event-data() -> ("OldVal"=w531:bool, "NewVal"=w532:bool)  [unwired: 1 in, 4 out]
        n331 = local write "Stopp"(w531) -> ()
      }
      event "Legende": Value Change {
        n332 = event-data() -> ()  [unwired: 1 in, 6 out]
        n333 = local read "PM-Graph"() -> (w536:cluster{dbl[], dbl[]}[])
        n334 = Array Size(array=w536) -> (size(s)=w535:i32)
        n335 = Max & Min(x=w535, y=2) -> (max(x,y)=w533:i32)  [unwired: 1 out]
        n336 = property on="PM-Graph" class="XYGraph (strikt)"("Legend Visible"="Legende", "LegNumRows"=w533) -> ()  [unwired: 2 in, 2 out]
      }
      event "PM-Graph": Mouse Move {
        w543 = 0
        n337 = event-data() -> ()  [unwired: 1 in, 5 out]
        n338 = property on="PM-Graph" class="XYGraph (strikt)"("Active Cursor"=w543) -> (error out=w556:errorcluster, "Cursor.Cursor Plot"=w542:i32, "Cursor.Cursor X"=w540:dbl, "Cursor.Cursor Index"=w541:i32)  [unwired: 2 in, 1 out]
        "n [1/min]" <- w540
        n339 = local read "AFR, EGT"() -> (w544:bool)
        n340 = case shown="True" w544 {
          tunnel: [w557 w568] -> w546
          tunnel: [w557 w565] -> w545
          tunnel: w541 -> [_ w564]
          tunnel: w542 -> [_ w561]
          frame False {
            w557 = 0.0
          }
          frame True {
            w559 = 2
            n341 = Quotient & Remainder(x=w561, y=w559) -> (floor(x/y)=w560:i32)  [unwired: 1 out]
            n342 = Multiply(x=w560, y=w559) -> (x*y=w558:i32)
            n343 = local read "AFR,EGT-Graph"() -> (w563:cluster{dbl[], "AFR":dbl[]}[])
            n344 = Increment(x=w558) -> (x+1=w562:i32)
            n345 = Index Array(array=w563, index=w558) -> (element=w569:cluster{dbl[], "AFR":dbl[]})
            n346 = Index Array(array=w563, index=w562) -> (element=w567:cluster{dbl[], "AFR":dbl[]})
            n347 = Unbundle(w569) -> ("AFR"=w570:dbl[])  [unwired: 1 out]
            n348 = Unbundle(w567) -> ("AFR"=w566:dbl[])  [unwired: 1 out]
            n349 = Index Array(array=w570, index=w564) -> (element=w568:dbl)
            n350 = Index Array(array=w566, index=w564) -> (element=w565:dbl)
          }
        }
        "AFR / l" <- w546
        "EGT [°C]" <- w545
        n351 = Quotient & Remainder(x=w542, y=2) -> (x-y*floor(x/y)=w547:i32)  [unwired: 1 out]
        n352 = property on="PM-Graph" class="XYGraph (strikt)"(error in=w556, "Active Plot"=w542) -> (error out=w538:errorcluster, "Plot.Plot Color"=w539:u32)  [unwired: 1 in, 1 out]
        n353 = Equal To 0?(x=w547) -> (x = 0?=w554:bool)
        n354 = property on="AFR,EGT-Graph" class="XYGraph (strikt)"(error in=w538, "Active Cursor"=w543, "Cursor.Cursor X"=w540, "Cursor.Cursor Color"=w539) -> ()  [unwired: 1 in, 2 out]
        n355 = property on="n [1/min]" class="DigWert (strikt)"("NumText.TextColor"=w539) -> ()  [unwired: 2 in, 2 out]
        n356 = property on="P [PS]" class="DigWert (strikt)"("NumText.TextColor"=w539) -> ()  [unwired: 2 in, 2 out]
        n357 = property on="M [Nm]" class="DigWert (strikt)"("NumText.TextColor"=w539) -> ()  [unwired: 2 in, 2 out]
        n358 = property on="AFR / l" class="DigWert (strikt)"("NumText.TextColor"=w539) -> ()  [unwired: 2 in, 2 out]
        n359 = property on="EGT [°C]" class="DigWert (strikt)"("NumText.TextColor"=w539) -> ()  [unwired: 2 in, 2 out]
        n360 = property on="PM-Graph" class="XYGraph (strikt)"(error in=w538, "Active Cursor"=w543, "Cursor.Cursor Color"=w539) -> ()  [unwired: 1 in, 2 out]
        n361 = local read "Übersetzung aus:"() -> (w551:T2)
        n362 = property on="PM-Graph" class="XYGraph (strikt)"("Active Cursor"=0) -> ("Cursor.Cursor Y"=w549:dbl, "Cursor.Cursor X"=w548:dbl)  [unwired: 2 in, 2 out]
        n363 = case shown="False" w554 {
          tunnel: [w577 w594] -> w553
          tunnel: [w576 w593] -> w552
          tunnel: w551 -> [w575 w597]
          tunnel: w549 -> [w574 w596]
          tunnel: w548 -> [w573 w595]
          tunnel: w541 -> [w571 w592]
          tunnel: w542 -> [w572 w591]
          frame False {
            n364 = case shown="\"Vario [km/h]\"" w575 {
              tunnel: [w580 w583] -> w577
              tunnel: [w579 w590] -> w576
              tunnel: w574 -> [w579 w590]
              tunnel: w573 -> [w578 _]
              tunnel: w572 -> [_ w585]
              tunnel: w571 -> [_ w584]
              frame Default {
                n365 = Multiply(x=w578, y=0.00014237924281946062) -> (x*y=w581:dbl)
                n366 = Multiply(x=w579, y=w581) -> (x*y=w580:dbl)
              }
              frame "Vario [km/h]" {
                n367 = Decrement(x=w585) -> (x-1=w588:i32)
                n368 = local read "PM-Graph"() -> (w589:cluster{dbl[], dbl[]}[])
                n369 = Index Array(array=w589, index=w588) -> (element=w587:cluster{dbl[], dbl[]})
                n370 = Unbundle(w587) -> (w586:dbl[])  [unwired: 1 out]
                n371 = Index Array(array=w586, index=w584) -> (element=w583:dbl)
              }
            }
          }
          frame True {
            n372 = case shown="Standard" w597 {
              tunnel: w596 -> [w599 w605]
              tunnel: w595 -> [w600 _]
              tunnel: [w599 w605] -> w594
              tunnel: [w598 w604] -> w593
              tunnel: w592 -> [_ w606]
              tunnel: w591 -> [_ w610]
              frame Default {
                w601 = 7023.495702024609  # 60/(2Pi) * W/PS
                n373 = Divide(x=w601, y=w600) -> (x/y=w602:dbl)
                n374 = Multiply(x=w599, y=w602) -> (x*y=w598:dbl)
              }
              frame "Vario [km/h]" {
                n375 = Increment(x=w610) -> (x+1=w608:i32)
                n376 = local read "PM-Graph"() -> (w609:cluster{dbl[], dbl[]}[])
                n377 = Index Array(array=w609, index=w608) -> (element=w607:cluster{dbl[], dbl[]})
                n378 = Unbundle(w607) -> (w603:dbl[])  [unwired: 1 out]
                n379 = Index Array(array=w603, index=w606) -> (element=w604:dbl)
              }
            }
          }
        }
        "M [Nm]" <- w552
        "P [PS]" <- w553
      }
      event "AFR, EGT": Value Change {
        w612 = 0
        n380 = event-data() -> ("NewVal"=w615:bool)  [unwired: 1 in, 5 out]
        n381 = case shown="False" w615 {
          tunnel: [645 430] -> w616
          tunnel: [w617 w619] -> w614
          frame False {
            w617 = 2  # Deaktivieren
          }
          frame True {
            w619 = 0  # Aktivieren
          }
        }
        n382 = property on="PM-Graph" class="XYGraph (strikt)"("Active Cursor"=w612) -> ("Cursor.Cursor X"=w613:dbl, "Cursor.Cursor Color"=w611:u32)  [unwired: 2 in, 2 out]
        n383 = property on="AFR,EGT-Graph" class="XYGraph (strikt)"("Active Cursor"=w612, "Cursor.Cursor X"=w613, "Cursor.Cursor Color"=w611) -> ()  [unwired: 2 in, 2 out]
        n384 = property on="PM-Graph" class="XYGraph (strikt)"("Height"=w616) -> ()  [unwired: 2 in, 2 out]
        n385 = property on="Lambda" class="Bool. (strikt)"("DisabledEnum"=w614) -> ()  [unwired: 2 in, 2 out]
        n386 = property on="AFR / l" class="DigWert (strikt)"("DisabledEnum"=w614) -> ()  [unwired: 2 in, 2 out]
        n387 = property on="EGT [°C]" class="DigWert (strikt)"("DisabledEnum"=w614) -> ()  [unwired: 2 in, 2 out]
      }
      event "Lambda": Value Change {
        n388 = event-data() -> ("NewVal"=w623:bool)  [unwired: 1 in, 5 out]
        n389 = property on="AFR,EGT-Graph" class="XYGraph (strikt)"() -> ("Value"=w622:cluster{dbl[], "AFR":dbl[]}[])  [unwired: 2 in, 2 out]
        n390 = Array Size "Anzahl Plots"(array=w622) -> (size(s)=w621:i32)
        n391 = for {
          N: w621 -> [_]
          tunnel: w623 -> [w628]
          i -> [w626]
          n392 = Quotient & Remainder(x=w626, y=2) -> (x-y*floor(x/y)=w625:i32)  [unwired: 1 out]
          n393 = Equal To 0? "AFR-Plot?"(x=w625) -> (x = 0?=w624:bool)
          n394 = case shown="True" w624 {
            tunnel: w628 -> [_ w634]
            tunnel: w626 -> [_ w630]
            frame False {
            }
            frame True {
              w633 = 0
              w636 = 14.7  # Lambda -->AFR
              w635 = 0.06802721088435375  # AFR --> Lambda
              n395 = case shown="False" w634 {
                tunnel: ["AFR" "l"] -> w653
                tunnel: ["Anwendung" "Symbol"] -> w652
                tunnel: [20.0 1.6] -> w651
                tunnel: [10.0 0.4] -> w654
                tunnel: [1 2] -> w650
                frame False {
                }
                frame True {
                }
              }
              n396 = local read "AFR,EGT-Graph"() -> (w629:cluster{dbl[], "AFR":dbl[]}[])
              n397 = Index Array(array=w629, index=w630) -> (element=w642:cluster{dbl[], "AFR":dbl[]})
              n398 = Unbundle(w642) -> (w637:dbl[], "AFR"=w640:dbl[])
              n399 = property on="AFR,EGT-Graph" class="XYGraph (strikt)"("ActYScl"=w633, "YScale.NameLbl.Text"=w653, "YScale.NameLbl.FontName"=w652, "YScale.Maximum"=w651, "YScale.Minimum"=w654, "YScale.Precision"=w650) -> ("Height"=w645:u32, "YScale.NameLbl.Width"=w644:u32, "Top"=w643:i32)  [unwired: 2 in, 2 out]
              n400 = Multiply(x=w635, y=w640) -> (x*y=w641:dbl[])
              n401 = Multiply(x=w636, y=w640) -> (x*y=w639:dbl[])
              n402 = Select(t=w641, s=w634, f=w639) -> (s? t:f=w638:dbl[])
              n403 = Bundle(w637, w638) -> (w632:cluster{dbl[], dbl[]})  [unwired: 1 in]
              n404 = Subtract(x=w645, y=w644) -> (x-y=w649:u32)
              n405 = Divide(x=w649, y=2) -> (x/y=w647:dbl)
              n406 = Add(x=w647, y=w643) -> (x+y=w646:dbl)
              n407 = Replace Array Subset(array=w629, new element=w632, index=w630) -> (w631:cluster{dbl[], "AFR":dbl[]}[])
              n408 = property on="AFR,EGT-Graph" class="XYGraph (strikt)"("ActYScl"=w633, "YScale.NameLbl.Top"=w646) -> ()  [unwired: 2 in, 2 out]
              n409 = property on="AFR,EGT-Graph" class="XYGraph (strikt)"("Value"=w631) -> ()  [unwired: 2 in, 2 out]
            }
          }
        }
      }
      event "PM-Graph": Scale Range Change {
        n410 = event-data() -> ()  [unwired: 1 in, 8 out]
        n411 = property on="PM-Graph" class="XYGraph (strikt)"() -> ("XScale.Minimum"=w666:dbl, "XScale.Maximum"=w665:dbl)  [unwired: 2 in, 2 out]
        n412 = property on="AFR,EGT-Graph" class="XYGraph (strikt)"("XScale.Minimum"=w666, "XScale.Maximum"=w665) -> ()  [unwired: 2 in, 2 out]
      }
      event "AFR,EGT-Graph": Scale Range Change {
        n413 = event-data() -> ()  [unwired: 1 in, 8 out]
        n414 = property on="AFR,EGT-Graph" class="XYGraph (strikt)"() -> ("XScale.Minimum"=w668:dbl, "XScale.Maximum"=w667:dbl)  [unwired: 2 in, 2 out]
        n415 = property on="PM-Graph" class="XYGraph (strikt)"("XScale.Minimum"=w668, "XScale.Maximum"=w667) -> ()  [unwired: 2 in, 2 out]
      }
      event "PM-Graph": Plot Attribute Change {
        n416 = event-data() -> ()  [unwired: 1 in, 8 out]
        n417 = for {
          N: 7 -> [_]
          i -> [w672]
          n418 = Multiply(x=w672, y=2) -> (x*y=w670:i32)
          n419 = Increment(x=w670) -> (x+1=w674:i32)
          n420 = property on="PM-Graph" class="XYGraph (strikt)"("Active Plot"=w670, "Active Plot"=w674) -> ("Plot.Visible?"=w676:bool, "Plot.Visible?"=w675:bool)  [unwired: 2 in, 2 out]
          n421 = Or(x=w676, y=w675) -> (x .or. y?=w673:bool)
          n422 = property on="AFR,EGT-Graph" class="XYGraph (strikt)"("Active Plot"=w670, "Plot.Visible?"=w673, "Active Plot"=w674, "Plot.Visible?"=w673) -> ()  [unwired: 2 in, 2 out]
        }
      }
    }
  }
  n423 = property on="PM-Graph" class="XYGraph (strikt)"("Legend Visible"=TRUE, "LegNumRows"=2) -> ()  [unwired: 2 in, 2 out]
  n424 = property on="Fensterbereich" class="Bereich"("Origin"=T4 {"Horizontal"=8, "Vertical"=6}) -> ()  [unwired: 2 in, 2 out]
  n425 = property on="AFR, EGT" class="Bool. (strikt)"("Val(Sgnl)"=w10) -> ()  [unwired: 2 in, 2 out]
  n426 = property on="Lambda" class="Bool. (strikt)"("Val(Sgnl)"=w10) -> ()  [unwired: 2 in, 2 out]
  n427 = property on="Fensterbereich" class="Bereich"("Origin"=T4 {"Horizontal"=8, "Vertical"=6}) -> ()  [unwired: 2 in, 2 out]
  n428 = property on="Überlagerung" class="Bool. (strikt)"("Value"=FALSE) -> ()  [unwired: 2 in, 2 out]
  n429 = case shown="True" "Berechnen" {
    selector: "Berechnen" -> [_ w680]
    frame False {
    }
    frame True {
      n430 = property on="Berechnen" class="Bool. (strikt)"("Value"=w680, "DisabledEnum"=T5."Enabled" ("Deaktiviert")) -> (error out=w677:errorcluster)  [unwired: 2 in, 1 out]
      n431 = property on="Öffnen" class="Bool. (strikt)"(error in=w677, "Val(Sgnl)"=TRUE ("Wert (signalisierend)")) -> ()  [unwired: 1 in, 2 out]
    }
  }
  n432 = property on="Berechnen" class="Bool. (strikt)"("DisabledEnum"=w22) -> ()  [unwired: 2 in, 2 out]
  n433 = property on="Überlagern" class="Bool. (strikt)"("DisabledEnum"=w22) -> ()  [unwired: 2 in, 2 out]
  n434 = property on="Speichern" class="Bool. (strikt)"("DisabledEnum"=w22) -> ()  [unwired: 2 in, 2 out]
  n435 = property on="Drucken" class="Bool. (strikt)"("DisabledEnum"=w22) -> ()  [unwired: 2 in, 2 out]
  n436 = Bundle(w19, w19) -> (w9:cluster{dbl[], dbl[]})  [unwired: 1 in]
  n437 = Build Array(w9, w9) -> (w8:cluster{dbl[], dbl[]}[])
  n438 = property on="PM-Graph" class="XYGraph (strikt)"("Value"=w8, "Active Cursor"=w18, "Cursor.Cursor Color"=w18) -> ()  [unwired: 2 in, 2 out]
  n439 = property on="AFR,EGT-Graph" class="XYGraph (strikt)"("Value"=w8) -> ()  [unwired: 2 in, 2 out]
  n440 = property on="M [Nm]" class="DigWert (strikt)"("Value"=w11) -> ()  [unwired: 2 in, 2 out]
  n441 = property on="n [1/min]" class="DigWert (strikt)"("Value"=w11) -> ()  [unwired: 2 in, 2 out]
  n442 = property on="P [PS]" class="DigWert (strikt)"("Value"=w11) -> ()  [unwired: 2 in, 2 out]
  n443 = property on="EGT [°C]" class="DigWert (strikt)"("Value"=w11) -> ()  [unwired: 2 in, 2 out]
  n444 = property on="AFR / l" class="DigWert (strikt)"("Value"=w11) -> ()  [unwired: 2 in, 2 out]
  n445 = Bundle(w14, w14, w14, w14, w14, w14, w14) -> (→"Strecken":cluster{dbl, dbl, dbl, dbl, dbl, dbl, dbl})  [unwired: 1 in]
  n446 = property on="Gl. Mittelwert" class="DigWert (strikt)"("DisabledEnum"=w16) -> ()  [unwired: 2 in, 2 out]
  n447 = property on="Differenzenquotient" class="DigWert (strikt)"("DisabledEnum"=w16) -> ()  [unwired: 2 in, 2 out]
  n448 = property on="Ergebnis" class="Str"("Value"=w13) -> ()  [unwired: 2 in, 2 out]
  n449 = property on="Pmax" class="Str"("Value"=w13) -> ()  [unwired: 2 in, 2 out]
  n450 = property on="Fahrzeugdaten" class="Str"("Value"=w13) -> ()  [unwired: 2 in, 2 out]
  n451 = property on="Dateiname" class="Str"("Value"=w13) -> ()  [unwired: 2 in, 2 out]
  n452 = property on="Überschrift Leistungsdiagramm" class="Str"("Value"=w13) -> ()  [unwired: 2 in, 2 out]
  n453 = property on="M [Nm]" class="DigWert (strikt)"("NumText.TextColor"=w12) -> ()  [unwired: 2 in, 2 out]
  n454 = property on="P [PS]" class="DigWert (strikt)"("NumText.TextColor"=w12) -> ()  [unwired: 2 in, 2 out]
  n455 = property on="n [1/min]" class="DigWert (strikt)"("NumText.TextColor"=w12) -> ()  [unwired: 2 in, 2 out]
  n456 = property on="AFR / l" class="DigWert (strikt)"("NumText.TextColor"=w12) -> ()  [unwired: 2 in, 2 out]
  n457 = property on="EGT [°C]" class="DigWert (strikt)"("NumText.TextColor"=w12) -> ()  [unwired: 2 in, 2 out]
  n458 = property on="Mv: M0 [Nm]" class="DigWert (strikt)"("DisabledEnum"=w16) -> ()  [unwired: 2 in, 2 out]
  n459 = property on="Mv: n1 [1/min]" class="DigWert (strikt)"("DisabledEnum"=w16) -> ()  [unwired: 2 in, 2 out]
  n460 = property on="Mv: M1 [Nm]" class="DigWert (strikt)"("DisabledEnum"=w16) -> ()  [unwired: 2 in, 2 out]
  n461 = property on="AFR,EGT-Graph" class="XYGraph (strikt)"("ActYScl"=w6, "YScale.ScaleFit"=w6, "YScale.Maximum"=20.0, "YScale.Minimum"=10.0, "ActYScl"=1, "YScale.ScaleFit"=w6, "YScale.Maximum"=800.0, "YScale.Minimum"=0.0, "XScale.ScaleFit"=w6, "Smooth Update"=TRUE) -> ()  [unwired: 2 in, 2 out]
